vi "hanwang_LLSE 2.vi"(4 "error in (no error)":errorcluster, 5 "b":cdb[](array[numeric]), 7 "A":cdb[][](array[numeric]) format="%0.2f") -> (0 "error out":errorcluster, 2 "mean square error":dbl, 3 "x.estimate":cdb[](array[numeric]))   [LabVIEW 2022 SP3]
uses:
  <vilib>/Analysis/baseanly.llb/Complex A x B.vi
  <vilib>/Analysis/baseanly.llb/Complex A x Vector.vi
  <vilib>/Analysis/7linalg.llb/Solve Complex Linear Equations (single right hand).vi
  <vilib>/Analysis/NI_AALBase.lvlib
  <vilib>/Analysis/NI_AALPro.lvlib
panel:
  out "Solution Vector":cdb[](array[numeric]) format="%.2f"
  out "transposed array":cdb[][](array[numeric])
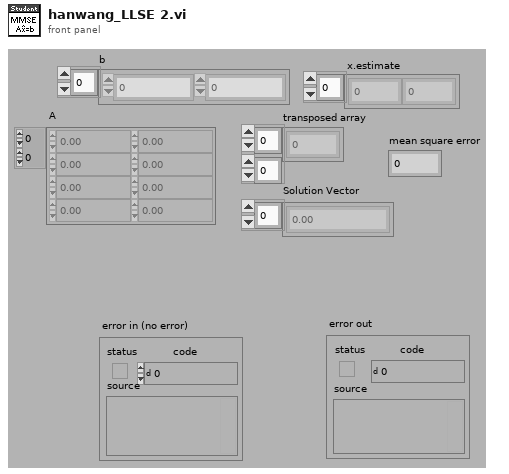
[diagram p1: front panel]
types:
  T1 = typedef "NI_Matrix.lvlib/ComplexMatrix.ctl" = cdb[][]
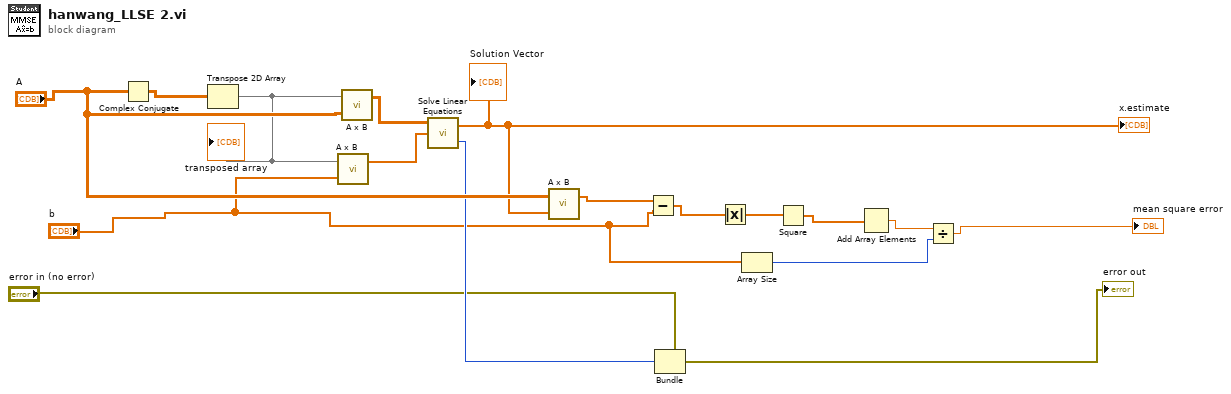
[diagram p0: block diagram]
diagram:
  n1 = Complex Conjugate(1:"A") -> (0:w17:cdb[][])
  n2 = Transpose 2D Array(2D array=w17) -> (transposed array=w2:cdb[][])
  "transposed array" <- w2
  n3 = call-poly <vilib>:"A x B.vi"("Vector"="b", "A"=w2) -> ("A x Vector"=w5:cdb[])  [unwired: 1 out]
  n4 = call-poly <vilib>:"A x B.vi"("B"="A", "A"=w2) -> ("A x B"=w4:T1)  [unwired: 1 out]
  n5 = call-poly <vilib>:"Solve Linear Equations.vi"("Known Vector"=w5, "Input Matrix"=w4) -> ("error"=w8:i32, "Solution Vector"=w1:cdb[])  [unwired: 1 in]
  "x.estimate" <- w1
  "Solution Vector" <- w1
  n6 = call-poly <vilib>:"A x B.vi"("Vector"=w1, "A"="A") -> ("A x Vector"=w15:cdb[])  [unwired: 1 out]
  n7 = Subtract ("Subtract.vi")(x=w15, y="b") -> (x-y=w14:cdb[])
  n8 = Bundle(cluster="error in (no error)", "code"=w8) -> (→"error out":errorcluster)  [unwired: 2 in]
  n9 = Absolute Value ("Absolute Value.vi")(x=w14) -> (abs(x)=w13:dbl[])
  n10 = Array Size(array="b") -> (size(s)=w10:i32)
  n11 = Square(x=w13) -> (x^2=w12:dbl[])
  n12 = Add Array Elements(numeric array=w12) -> (sum=w11:dbl)
  n13 = Divide(x=w11, y=w10) -> (x/y=→"mean square error":dbl)
